vi "MRC Initialize All.vi"(8 "error out 2":errorcluster) -> (0 "error out":errorcluster)   [LabVIEW 2023]
uses:
  <vilib>/MRC/MrcLib.lvlib
  MrcLib.so
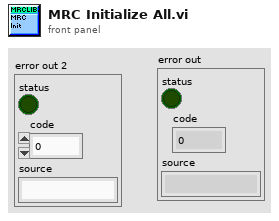
[diagram p1: front panel]
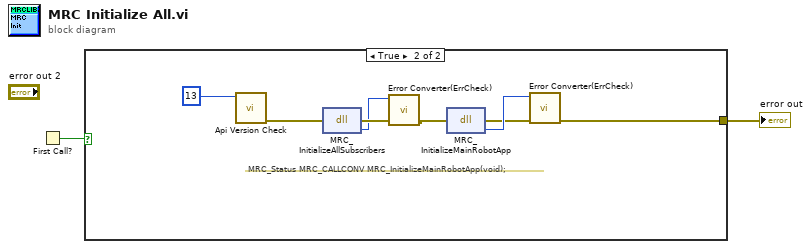
[diagram p0: block diagram]
diagram:
  n1 = First Call?() -> (First Call?: T/F=w2:bool)
  n2 = case shown="True" w2 {
    tunnel: [_ w8] -> w1
    frame False {
    }
    frame True {
      # "MRC_Status MRC_CALLCONV MRC_InitializeMainRobotApp(void);"
      n3 = call <vilib>:"Api Version Check.vi"("version"=u32 13) -> ("error out"=w6:errorcluster)  [unwired: 10 in]
      n4 = dll-call lib="MrcLib.*" fn="MRC_InitializeAllSubscribers"(error in=w6) -> (error out=w4:errorcluster, "return type"=w3:i32)  [unwired: 2 in, 1 out]
      n5 = call <vilib>:"Error Converter(ErrCheck).vi"("error in (no error)"=w4, "status"=w3) -> ("error out"=w5:errorcluster)  [unwired: 9 in]
      n6 = dll-call lib="MrcLib.*" fn="MRC_InitializeMainRobotApp"(error in=w5) -> (error out=w9:errorcluster, "return type"=w10:i32)  [unwired: 2 in, 1 out]
      n7 = call <vilib>:"Error Converter(ErrCheck).vi"("error in (no error)"=w9, "status"=w10) -> ("error out"=w8:errorcluster)  [unwired: 9 in]
    }
  }
  "error out" <- w1
